vi "Initialize Qeue.vi"(8 "error in (no error)":errorcluster, 10 "TCS COM Port":string="COM1", 11 "TCS in":refnum<class "TCS.lvclass">) -> (0 "error out":errorcluster, 3 "TCS out":refnum<class "TCS.lvclass">)   [LabVIEW 2018, in "TCS.lvclass"]
uses:
  TCS.lvclass
  TCS.lvclass/TCS.ctl
  RxTx/RxTx.lvclass
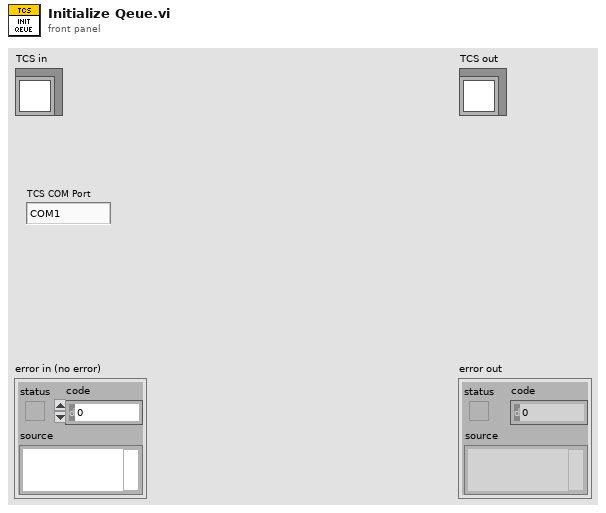
[diagram p1: front panel]
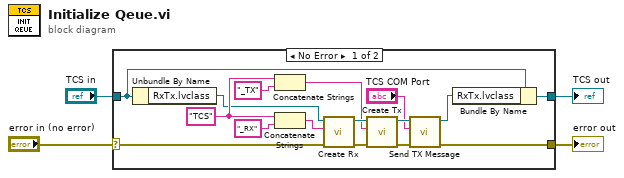
[diagram p0: block diagram]
diagram:
  n1 = case shown="No Error" "error in (no error)" {
    selector: "error in (no error)" -> [w15 w22]
    tunnel: [w7 w22] -> w2
    tunnel: [w19 w21] -> w1
    tunnel: "TCS in" -> [w20 w21]
    frame No Error {
      w16 = "TCS"
      n2 = Unbundle By Name(w20) -> ("RxTx.lvclass"=w14:refnum<class "RxTx.lvclass">)
      n3 = Concatenate Strings(w16, "_TX") -> (w10:string)
      n4 = Concatenate Strings(w16, "_RX") -> (w13:string)
      n5 = call "Create Rx.vi"("error in (no error)"=w15, "Reader Name"=w13, "RxTx in"=w14) -> ("error out"=w11:errorcluster, "RxTx out"=w12:refnum<class "RxTx.lvclass">)  [unwired: 7 in]
      n6 = call "Create Tx.vi"("error in (no error)"=w11, "Writer Name"=w10, "RxTx in"=w12) -> ("error out"=w6:errorcluster, "RxTx out"=w9:refnum<class "RxTx.lvclass">)  [unwired: 7 in]
      n7 = call "Send TX Message.vi"("error in (no error)"=w6, "element"="TCS COM Port", "RxTx in"=w9) -> ("error out"=w7:errorcluster, "RxTx out"=w8:refnum<class "RxTx.lvclass">)  [unwired: 7 in]
      n8 = Bundle By Name(cluster=w20, "RxTx.lvclass"=w8) -> (w19:refnum<class "TCS.lvclass">)
    }
    frame Error {
    }
  }
  "error out" <- w2
  "TCS out" <- w1
